vi "Consumer.vi"(8 "error in (no error)":errorcluster, 9 "Data":variant, 10 "Case ID":string, 11 "uService Template in":refnum<class "TCP Server.lvclass">) -> (0 "error out":errorcluster, 3 "uService Template out":refnum<class "TCP Server.lvclass">)   [LabVIEW 2020, in "TALOS.lvlib" / "TCP Server.lvlib" / "TCP Server.lvclass"]
uses:
  TCP Server.lvclass
  C:/LabVIEW Code/TALOS/talos/Father of all uServices/Father of all uServices/Father of all uServices.lvclass
  TCP Server Consumer Case Selector.ctl
  Ancestor/Ancestor/Ancestor.lvclass/Ancestor.ctl
  TCP Server.lvclass/TCP Server.ctl
  Father of all uServices/Father of all uServices Messages/Consumer Msg/Consumer Msg.lvclass/Consumer Msg.ctl
  Father of all uServices/Father of all uServices/Father of all uServices.lvclass/Father of all uServices.ctl
  Support VIs/Circus Config Param - Core.vi
  Support VIs/Generate Error.vi
  Father of all uServices/Father of all uServices/Children Methods/Update GUI.vi
  Support VIs/Circus Root Path.vi
  Support VIs/TALOS Config Param.vi
  FGV/Error Memory/Get Error Description.vi
  Ancestor/Ancestor/Read ID.vi
  Support VIs/Get Class Name.vi
  FGV/Error Memory/Error Memory Core.vi
  <vilib>/AdvancedString/Delimited String to 1D String Array.vi
  FGV/Error Memory/Error Crt Lvl checker.vi
  FGV/Error Memory/Error Memory Core.vi/40c8088d-b597-4017-91af-faa98e00292e.vi
  FGV/Error Memory/Error Memory Core.vi/d4a3ab98-063c-4e44-b43d-fbdcfe6c2be2.vi
  Father of all uServices/Father of all uServices/Father of all uServices.lvclass
  C:/LabVIEW Code/TALOS/builds/Actor Framework PPL/Actor Framework.lvlibp/1abvi3w/vi.lib/ActorFramework/Actor/Actor.lvclass
  Support VIs/Global Constants.vi
  Support VIs/Global Memory.vi
  <vilib>/Utility/LVClass/Get LV Class Name.vi
  Support VIs/Is in Packed Library.vi
  Support VIs/TALOS Root path.vi
  Support VIs/Read CSV worksheet.vi
  <vilib>/Utility/error.llb/General Error Handler.vi
  <vilib>/Utility/config.llb/Open Config Data.vi
  <vilib>/Utility/config.llb/Get Section Names.vi
  <vilib>/Utility/config.llb/Get Key Names.vi
  <vilib>/Utility/config.llb/Read Key.vi
  <vilib>/Utility/config.llb/Read Key (String).vi
  <vilib>/Utility/config.llb/Close Config Data.vi
  Guardian/Guardian/Extract list from Project INI file entry.vi
  Support VIs/Error Log.vi
  builds/Actor Framework PPL/Actor Framework.lvlibp/1abvi3w/vi.lib/ActorFramework/Actor/Read Self Enqueuer.vi
  <userlib>/_OpenG.lib/lvdata/lvdata.llb/Get Strings from Enum__ogtk.vi
  builds/Actor Framework PPL/Actor Framework.lvlibp/1abvi3w/vi.lib/ActorFramework/Message Enqueuer/Enqueue.vi
  Father of all uServices/Father of all uServices/Children Methods/Get GUI Item Value - String.vi
  Father of all uServices/Father of all uServices/Multiline string updater.vi
  Ancestor/Ancestor/Ancestor.lvclass
  <vilib>/Comparison/Equal/Equal Functor/Equal Functor.lvclass
  Father of all uServices/Father of all uServices Messages/Consumer Msg/Consumer Msg.lvclass
  TALOS.lvlib
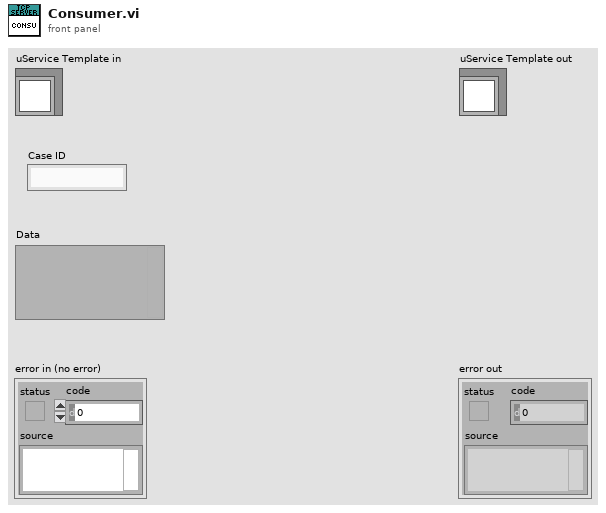
[diagram p1: front panel]
types:
  T1 = typedef "TALOS.lvlib/TCP Server.lvlib/TCP Server.lvclass/TCP Server Consumer Case Selector.ctl" = enum16{"Init", "Open Connection"}
  T2 = enum16{"Standard", "Buffered", "CRLF", "Immediate"}
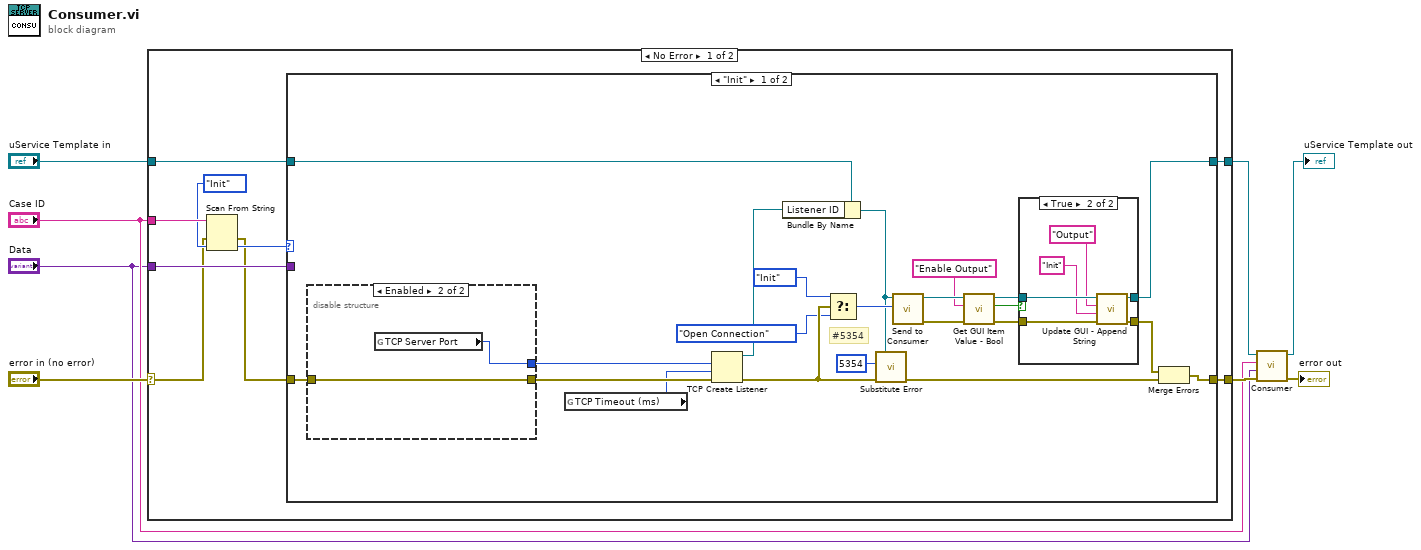
[diagram p0: block diagram]
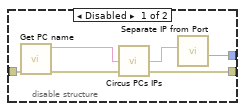
[diagram p2: hidden frame]
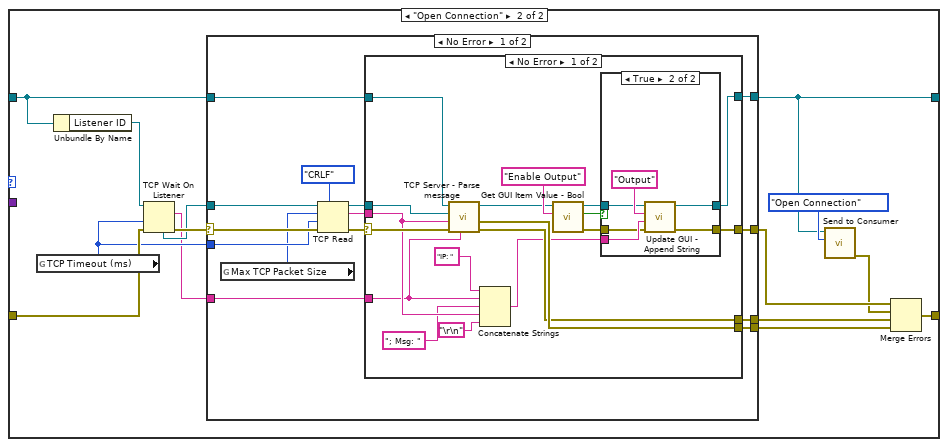
[diagram p4: hidden frame]
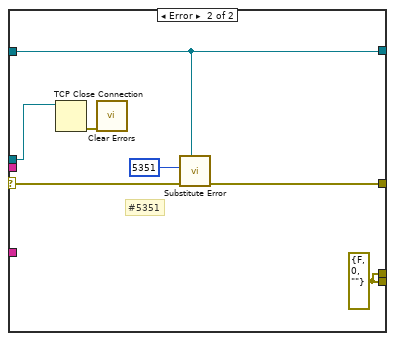
[diagram p6: hidden frame]
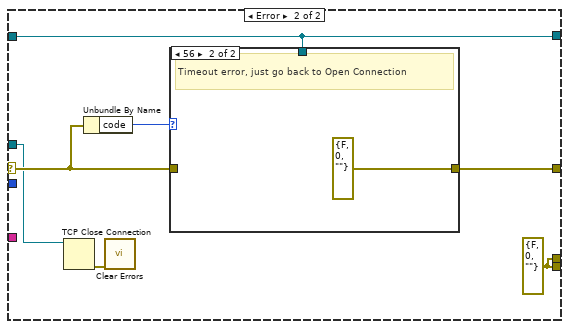
[diagram p7: hidden frame]
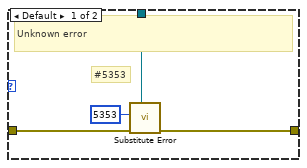
[diagram p8: hidden frame]
diagram:
  n1 = case shown="No Error" "error in (no error)" {
    selector: "error in (no error)" -> [w10 w129]
    tunnel: "uService Template in" -> [w16 w130]
    tunnel: [w14 w130] -> w4
    tunnel: [w15 w129] -> w3
    tunnel: "Case ID" -> [w13 _]
    tunnel: "Data" -> [w17 _]
    frame No Error {
      n2 = Scan From String(input string=w13, error in=w10, default 1=TCP_Server_Consumer_Case_Selector."Init") -> (error out=w9:errorcluster, output 1=w11:T1)  [unwired: 2 in, 2 out]
      n3 = case shown="\"Init\"" w11 {
        tunnel: w17 -> [_ _]
        tunnel: w9 -> [w21 w65]
        tunnel: w16 -> [w35 w60]
        tunnel: [w33 w62] -> w15
        tunnel: [w29 w61] -> w14
        frame "Init" {
          # "#5354"
          n4 = disable-structure shown="Enabled" {
            disable-tunnel: w21 -> [w45 w46]
            disable-tunnel: [w42 w46] -> w20
            disable-tunnel: [w41 w47] -> w19
            frame Disabled {
              n5 = call "Get PC name.vi"("error in (no error)"=w45) -> ("error out"=w44:errorcluster, "Hostname"=w40:string)  [unwired: 9 in]
              n6 = call "Circus PCs IPs.vi"("error in (no error)"=w44, "ID"=w40) -> ("error out"=w42:errorcluster, "IP"=w43:string)  [unwired: 2 in]
              n7 = call "Separate IP from Port.vi"("IP+Port"=w43) -> ("Port"=w41:u16)  [unwired: 9 in, 1 out]
            }
            frame Enabled {
              n8 = global read "Global Constants.vi" "TCP Server Port"() -> (w47:u16)
            }
          }
          n9 = global read "Global Constants.vi" "TCP Timeout (ms)"() -> (w18:i32)
          n10 = TCP Create Listener(8:w20, 9:w18, 10:w19) -> (0:w39:errorcluster, 3:w34:refnum<k5>)  [unwired: 2 in, 1 out]
          n11 = Bundle By Name(cluster=w35, "Listener ID"=w34) -> (w31:refnum<class "TCP Server.lvclass">)
          n12 = Select(t=TCP_Server_Consumer_Case_Selector."Init", s=w39, f=TCP_Server_Consumer_Case_Selector."Open Connection") -> (s? t:f=w36:T1)
          n13 = call "Substitute Error.vi"("LabVIEW Object"=w31, "error in (no error)"=w39, "Error Code"=5354) -> ("error out"=w32:errorcluster)  [unwired: 8 in]
          n14 = call "Send to Consumer.vi"("Case ID"=w36, "uService Template in"=w31) -> ("error out"=w26:errorcluster, "uService Template out"=w27:refnum<class "TCP Server.lvclass">)  [unwired: 8 in]
          n15 = call "Get GUI Item Value - Bool.vi"("error in (no error)"=w26, "FP Item Name"="Enable Output" ("Parameter Name"), "uService Template in"=w27) -> ("error out"=w25:errorcluster, "Value"=w24:bool, "uService Template out"=w23:refnum<class "TCP Server.lvclass">)  [unwired: 6 in]
          n16 = case shown="True" w24 {
            tunnel: w23 -> [w49 w55]
            tunnel: [w49 w54] -> w29
            tunnel: [w48 w53] -> w28
            tunnel: w25 -> [w48 w50]
            frame False {
            }
            frame True {
              n17 = call "Update GUI - Append String.vi"("error in (no error)"=w50, "String"="Init", "GUI Item Name"="Output", "Father of all uServices in"=w55) -> ("error out"=w53:errorcluster, "Father of all uServices out"=w54:refnum<class "TCP Server.lvclass">)  [unwired: 6 in]
            }
          }
          n18 = Merge Errors(w28, w32) -> (w33:errorcluster)
        }
        frame "Open Connection" {
          n19 = global read "Global Constants.vi" "TCP Timeout (ms)"() -> (w59:i32)
          n20 = Unbundle By Name(w60) -> ("Listener ID"=w66:refnum<k5>)
          n21 = TCP Wait On Listener(8:w65, 9:w59, 11:w66) -> (0:w69:errorcluster, 2:w58:string, 4:w68:refnum<k5>)  [unwired: 1 in, 2 out]
          n22 = case shown="No Error" w69 {
            selector: w69 -> [w83 w121]
            tunnel: w68 -> [w82 w118]
            tunnel: [w77 w122] -> w64
            tunnel: w60 -> [w76 w120]
            tunnel: [w75 w120] -> w61
            tunnel: w59 -> [w74 _]
            tunnel: w58 -> [w72 _]
            tunnel: [w71 w119] -> w57
            tunnel: [w70 w119] -> w56
            frame No Error {
              n23 = global read "Global Constants.vi" "Max TCP Packet Size"() -> (w73:i32)
              n24 = TCP Read(connection ID=w82, bytes to read=w73, error in (no error)=w83, 7:T2."CRLF" ("mode (standard)"), 9:w74) -> (connection ID out=w79:refnum<k5>, data out=w78:string, error out=w80:errorcluster)
              n25 = case shown="No Error" w80 {
                selector: w80 -> [w101 w115]
                tunnel: w79 -> [w99 w110]
                tunnel: w78 -> [w97 _]
                tunnel: [w96 w114] -> w77
                tunnel: w76 -> [w100 w113]
                tunnel: [w95 w113] -> w75
                tunnel: w72 -> [w86 _]
                tunnel: [w87 w112] -> w71
                tunnel: [w85 w112] -> w70
                frame No Error {
                  n26 = call "TCP Server - Parse message.vi"("Sender IP"=w86, "error in (no error)"=w101, "Message"=w97, "TCP Client ID"=w99, "TCP Server in"=w100) -> ("error out"=w85:errorcluster, "External error out"=w87:errorcluster, "TCP Server out"=w89:refnum<class "TCP Server.lvclass">)  [unwired: 4 in]
                  n27 = Concatenate Strings("IP: " ("string"), w86, "; Msg: " ("string"), w97, "\r\n") -> (w84:string)
                  n28 = call "Get GUI Item Value - Bool.vi"("FP Item Name"="Enable Output" ("Parameter Name"), "uService Template in"=w89) -> ("error out"=w91:errorcluster, "Value"=w90:bool, "uService Template out"=w88:refnum<class "TCP Server.lvclass">)  [unwired: 7 in]
                  n29 = case shown="True" w90 {
                    tunnel: [w102 w109] -> w96
                    tunnel: [w103 w106] -> w95
                    tunnel: w88 -> [w103 w107]
                    tunnel: w84 -> [_ w105]
                    tunnel: w91 -> [w102 w104]
                    frame False {
                    }
                    frame True {
                      n30 = call "Update GUI - Append String.vi"("error in (no error)"=w104, "String"=w105, "GUI Item Name"="Output", "Father of all uServices in"=w107) -> ("error out"=w109:errorcluster, "Father of all uServices out"=w106:refnum<class "TCP Server.lvclass">)  [unwired: 6 in]
                    }
                  }
                }
                frame Error {
                  w112 = errorcluster {"status"=FALSE, "code"=0, "source"=""} ("External error out")
                  # "#5351"
                  n31 = TCP Close Connection(connection ID=w110) -> (error out=w111:errorcluster)  [unwired: 2 in, 1 out]
                  n32 = call <vilib>:"Clear Errors.vi"("error in (no error)"=w111) -> ()  [unwired: 5 in, 2 out]
                  n33 = call "Substitute Error.vi"("LabVIEW Object"=w113, "error in (no error)"=w115, "Error Code"=5351) -> ("error out"=w114:errorcluster)  [unwired: 8 in]
                }
              }
            }
            frame Error {
              w119 = errorcluster {"status"=FALSE, "code"=0, "source"=""} ("External error out")
              n34 = TCP Close Connection(connection ID=w118) -> (error out=w117:errorcluster)  [unwired: 2 in, 1 out]
              n35 = Unbundle By Name(w121) -> ("code"=w123:i32)
              n36 = call <vilib>:"Clear Errors.vi"("error in (no error)"=w117) -> ()  [unwired: 5 in, 2 out]
              n37 = case shown="56" w123 {
                tunnel: [w126 errorcluster {"status"=FALSE, "code"=0, "source"=""} ("error IO")] -> w122
                tunnel: w121 -> [w127 _]
                tunnel: w120 -> [w125 _]
                frame Default {
                  # "#5353"
                  # "Unknown error"
                  n38 = call "Substitute Error.vi"("LabVIEW Object"=w125, "error in (no error)"=w127, "Error Code"=5353) -> ("error out"=w126:errorcluster)  [unwired: 8 in]
                }
                frame 56 {
                  # "Timeout error, just go back to Open Connection"
                }
              }
            }
          }
          n39 = call "Send to Consumer.vi"("Case ID"=TCP_Server_Consumer_Case_Selector."Open Connection", "uService Template in"=w61) -> ("error out"=w63:errorcluster)  [unwired: 8 in, 1 out]
          n40 = Merge Errors(w64, w63, w56, w57) -> (w62:errorcluster)
        }
      }
    }
    frame Error {
    }
  }
  n41 = call-parent "Consumer.vi"("error in (no error)"=w3, "Data"="Data", "Case ID"="Case ID", "uService Template in"=w4) -> ("error out"=→"error out":errorcluster, "uService Template out"=→"uService Template out":refnum<class "TCP Server.lvclass">)  [unwired: 6 in]
